vi "Open.vi"(3 "Timeout":u32=2000, 4 "Addr":string="[C:DSO][D:DSO-X][T:USB][PID:0x5537][VID:0x4348][EI:0x82][EO:0x2][CFG:1][I:0]", 5 "UCI_DllPath":path) -> (0 "error_out":errorcluster caption="错误输出", 1 "ResultDescription":string, 2 "Session_id":i32)   [LabVIEW 2015]
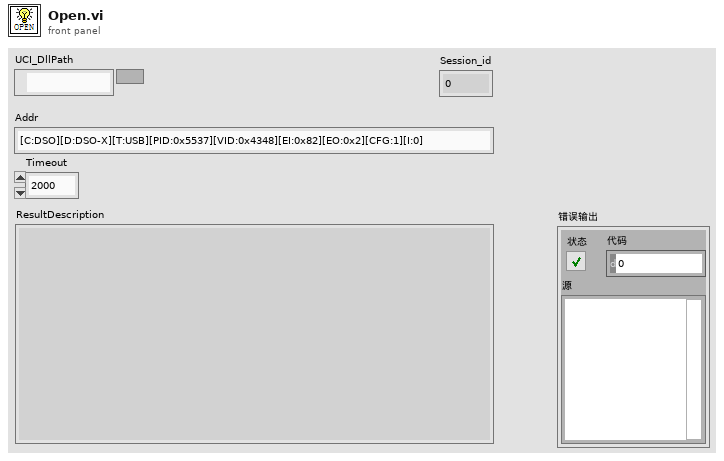
[diagram p1: front panel]
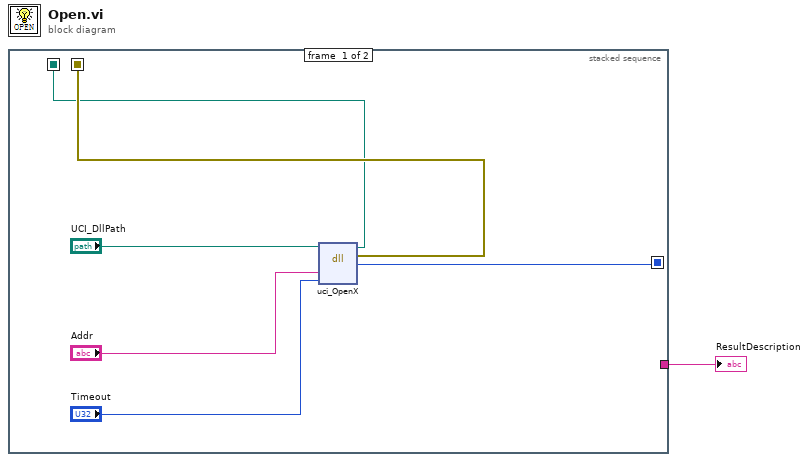
[diagram p0: block diagram]
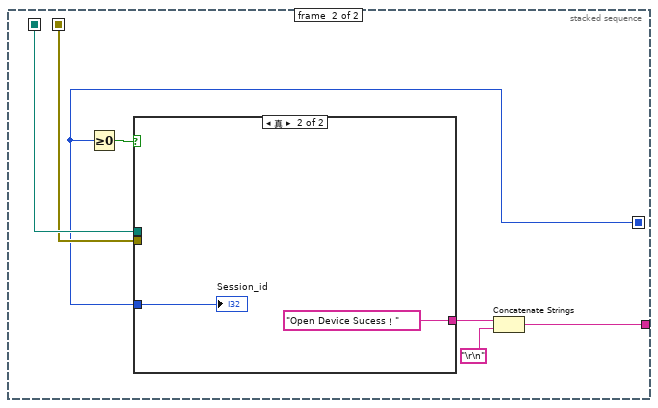
[diagram p2: hidden frame]
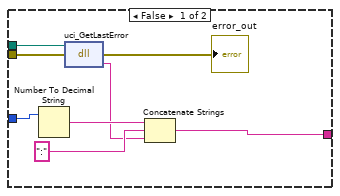
[diagram p3: hidden frame]
diagram:
  n1 = stacked-sequence {
    seq-local: [w5 _] -> [_ w11]
    seq-local: [w3 _] -> [_ w13]
    seq-local: [w4 _] -> [_ w12]
    tunnel: [_ w8] -> w1
    frame #0 {
      n2 = dll-call lib="E:/JL-Project/LabView-Project/ASCII/uci.dll" fn="uci_OpenX"(path in="UCI_DllPath", "_addr"="Addr", "_timeout"="Timeout") -> (path out=w3:path, error out=w4:errorcluster, "返回类型"=w5:i32)  [unwired: 4 in]
    }
    frame #1 {
      n3 = Greater Or Equal To 0?(x=w11) -> (x >= 0?=w14:bool)
      n4 = case shown="真" w14 {
        tunnel: w13 -> [w22 _]
        tunnel: w12 -> [w21 _]
        tunnel: w11 -> [w19 w24]
        tunnel: [w15 "Open Device Sucess！"] -> w9
        frame False {
          n5 = Number To Decimal String(number=w19) -> (decimal integer string=w18:string)  [unwired: 1 in]
          n6 = dll-call lib="E:/JL-Project/LabView-Project/ASCII/uci.dll" fn="uci_GetLastError"(path in=w22, error in=w21) -> (error out=→"error_out":errorcluster, "返回类型"=w16:string)  [unwired: 1 in, 1 out]
          n7 = Concatenate Strings(w18, ":" ("字符串"), w16) -> (w15:string)
        }
        frame True {
          "Session_id" <- w24
        }
      }
      n8 = Concatenate Strings(w9, "\r\n") -> (w8:string)
    }
  }
  "ResultDescription" <- w1
